vi "TestDriveEncoders.vi"(2 "WheelDiameter(in)":dbl=4.0, 3 "CountsPerRevolution":i32=4096, 4 "ZeroSensors":bool, 5 "RobotDriveMotors":T4[](array[typedef])) -> (0 "Drive Encoder Outputs":T3, 1 "Drive Encoder Outputs Raw":T1)   [LabVIEW 2017]
uses:
  <vilib>/Rock Robotics/WPI/MotorControl/WPI_MotorControlDeviceRef.ctl
  <vilib>/Rock Robotics/WPI/MotorControl/WPI_MotorControlType.ctl
  <vilib>/Rock Robotics/SystemInterfaces/DIO/FPGA_DIOPWMChannel.ctl
  <vilib>/Rock Robotics/WPI/PWM/WPI_PWMDeadband.ctl
  <vilib>/Rock Robotics/SystemInterfaces/DIO/FPGA_DIOChannel.ctl
  ArgosLib/Drive/MotorControl/TypeDefs/RobotDriveMotorSelectorEnum.ctl
  <vilib>/Rock Robotics/WPI/ThirdParty/Phoenix-LabVIEW/Motor Controller/Get/CTRE_Phoenix_MotorController_GetSelectedSensorData.vi
  ArgosLib/ArgosLib.lvlib
panel:
  out "Other Encoder Outputs":T2
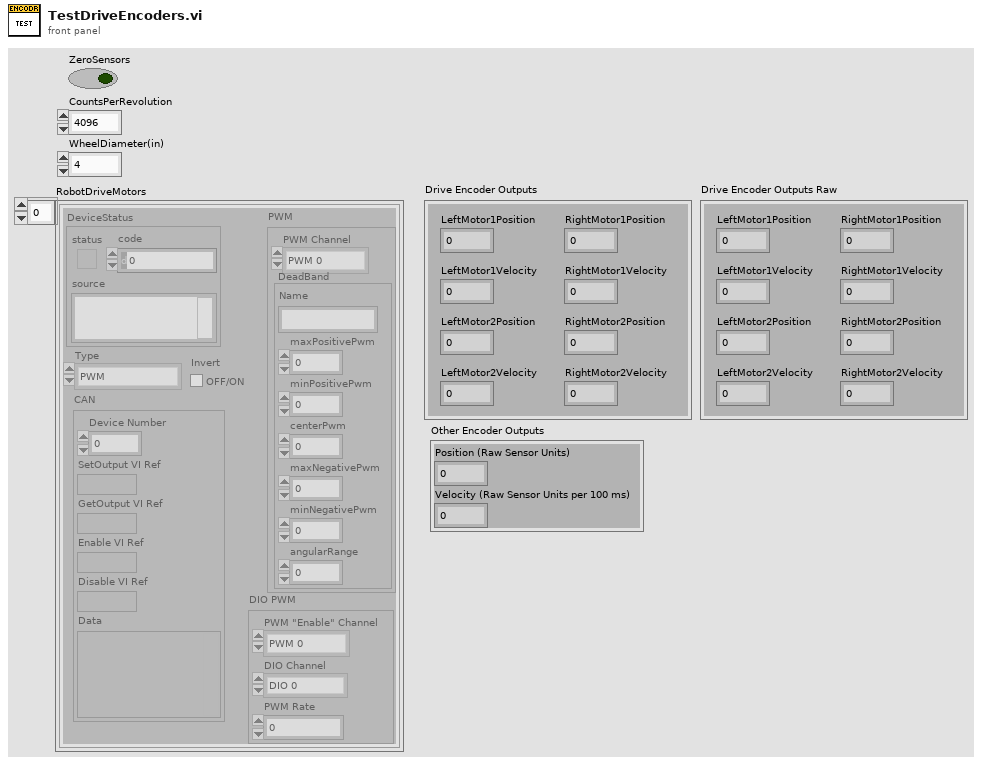
[diagram p1: front panel]
types:
  T1 = cluster{"LeftMotor1Position ":i32, "LeftMotor1Velocity":i32, "RightMotor1Velocity ":i32, "RightMotor1Position ":i32, "LeftMotor2Position ":i32, "LeftMotor2Velocity ":i32, "RightMotor2Position":i32, "RightMotor2Velocity":i32}
  T2 = cluster{"Position (Raw Sensor Units)":i32, "Velocity (Raw Sensor Units per 100 ms)":i32}
  T3 = cluster{"LeftMotor1Position ":dbl, "LeftMotor1Velocity":dbl, "RightMotor1Velocity ":dbl, "RightMotor1Position ":dbl, "LeftMotor2Position ":dbl, "LeftMotor2Velocity ":dbl, "RightMotor2Position":dbl, "RightMotor2Velocity":dbl}
  T4 = typedef "WPI_MotorControlDeviceRef.ctl" = cluster{"DeviceStatus":errorcluster, "Type":T5, "PWM":cluster{"PWM Channel":T6, "DeadBand":T7}, "CAN":cluster{"Device Number":u8, "SetOutput VI Ref":variant, "GetOutput VI Ref":variant, "Enable VI Ref":variant, "Disable VI Ref":variant, "Data":variant}, "Invert":bool, "DIO PWM":cluster{"PWM \"Enable\" Channel":T6, "DIOChannel":T8, "PWM Rate":dbl}}
  T5 = typedef "WPI_MotorControlType.ctl" = enum16{"PWM", "CAN", "DIO PWM"}
  T6 = typedef "FPGA_DIOPWMChannel.ctl" = enum8{"PWM 0", "PWM 1", "PWM 2", "PWM 3", "PWM 4", "PWM 5", "PWM 6", "PWM 7", "PWM 8", "PWM 9", "PWM MXP 0", "PWM MXP 1", "PWM MXP 2", "PWM MXP 3", "PWM MXP 4", "PWM MXP 5", "PWM MXP 6", "PWM MXP 7", "PWM MXP 8", "PWM MXP 9", "Invalid"}
  T7 = typedef "WPI_PWMDeadband.ctl" = cluster{"Name":string, "maxPositivePwm":i32, "minPositivePwm":i32, "centerPwm":i32, "maxNegativePwm":i32, "minNegativePwm":i32, "angularRange":u16}
  T8 = typedef "FPGA_DIOChannel.ctl" = enum8{"DIO 0", "DIO 1", "DIO 2", "DIO 3", "DIO 4", "DIO 5", "DIO 6", "DIO 7", "DIO 8", "DIO 9", "DIO MXP 0", "DIO MXP 1", "DIO MXP 2", "DIO MXP 3", "DIO MXP 4", "DIO MXP 5", "DIO MXP 6", "DIO MXP 7", "DIO MXP 8", "DIO MXP 9", "DIO MXP 10", "DIO MXP 11", "DIO MXP 12", "DIO MXP 13", "DIO MXP 14", "DIO MXP 15", "SPI Port CS1", "SPI Port CS2", "SPI Port CS3", "SPI Port MISO", "SPI Port MOSI", "Invalid"}
  T9 = typedef "ArgosLib.lvlib/RobotDriveMotorSelectorEnum.ctl" = enum16{"Left Motor 1", "Right Motor 1", "Left Motor 2", "Right Motor 2", "Left Motor 3", "Right Motor 3"}
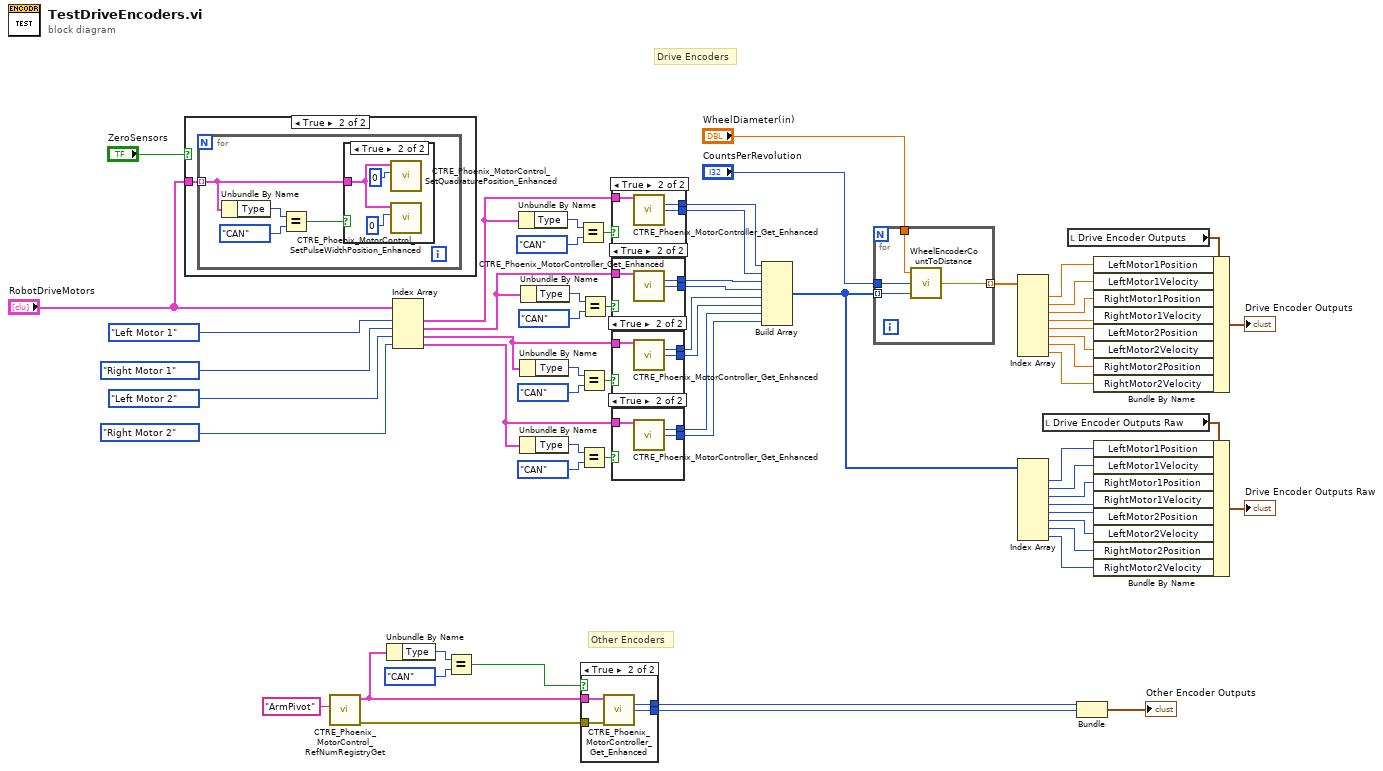
[diagram p0: block diagram]
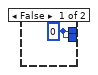
[diagram p2: hidden frame]
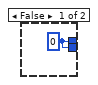
[diagram p3: hidden frame]
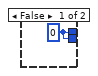
[diagram p4: hidden frame]
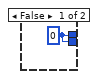
[diagram p5: hidden frame]
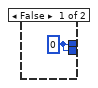
[diagram p6: hidden frame]
diagram:
  # "Other Encoders"
  # "Drive Encoders"
  n1 = case shown="True" "ZeroSensors" {
    tunnel: "RobotDriveMotors" -> [_ w64]
    frame False {
    }
    frame True {
      n2 = for {
        tunnel: w64 -> [w68] mode=indexing
        n3 = Unbundle By Name(w68) -> ("Type"=w67:T5)
        n4 = Equal?(x=w67, y=WPI_MotorControlType."CAN" ("Type")) -> (x = y?=w65:bool)
        n5 = case shown="True" w65 {
          tunnel: w68 -> [_ w69]
          frame False {
          }
          frame True {
            n6 = call <vilib>:"CTRE_Phoenix_MotorControl_SetQuadraturePosition_Enhanced.vi"("New Position"=0, "PhoenixMotorControlDevRef"=w69) -> ()  [unwired: 8 in, 2 out]
            n7 = call <vilib>:"CTRE_Phoenix_MotorControl_SetPulseWidthPosition_Enhanced.vi"("New Position"=0, "PhoenixMotorControlDevRef"=w69) -> ()  [unwired: 8 in, 2 out]
          }
        }
      }
    }
  }
  n8 = call <vilib>:"CTRE_Phoenix_MotorControl_RefNumRegistryGet.vi"("refnum name"="ArmPivot") -> ("error out"=w37:errorcluster, "PhoenixMotorControlDevRef"=w18:T4)  [unwired: 9 in]
  n9 = Unbundle By Name(w18) -> ("Type"=w19:T5)
  n10 = Index Array(array="RobotDriveMotors", index #1=RobotDriveMotorSelectorEnum."Left Motor 1" ("Motor Selector Enum"), index #2=RobotDriveMotorSelectorEnum."Right Motor 1" ("Motor Selector Enum"), index #3=RobotDriveMotorSelectorEnum."Left Motor 2" ("Motor Selector Enum"), index #4=RobotDriveMotorSelectorEnum."Right Motor 2" ("Motor Selector Enum")) -> (element #1=w8:T4, element #2=w7:T4, element #3=w6:T4, element #4=w5:T4)
  n11 = Equal?(x=w19, y=WPI_MotorControlType."CAN" ("Type")) -> (x = y?=w17:bool)
  n12 = Unbundle By Name(w8) -> ("Type"=w16:T5)
  n13 = Unbundle By Name(w6) -> ("Type"=w12:T5)
  n14 = Unbundle By Name(w5) -> ("Type"=w9:T5)
  n15 = Unbundle By Name(w7) -> ("Type"=w13:T5)
  n16 = Equal?(x=w16, y=WPI_MotorControlType."CAN" ("Type")) -> (x = y?=w1:bool)
  n17 = Equal?(x=w12, y=WPI_MotorControlType."CAN" ("Type")) -> (x = y?=w3:bool)
  n18 = Equal?(x=w9, y=WPI_MotorControlType."CAN" ("Type")) -> (x = y?=w4:bool)
  n19 = Equal?(x=w13, y=WPI_MotorControlType."CAN" ("Type")) -> (x = y?=w2:bool)
  n20 = case shown="True" w17 {
    tunnel: w37 -> [_ w76]
    tunnel: [w72 w75] -> w36
    tunnel: [w72 w74] -> w35
    tunnel: w18 -> [_ w73]
    frame False {
      w72 = 0 ("Position (Raw Sensor Units)")
    }
    frame True {
      n21 = call-poly <vilib>:"CTRE_Phoenix_MotorController_Get_Enhanced.vi"("PhoenixMotorControlDevRef"=w73, "error in"=w76) -> ("Position (Raw Sensor Units)"=w75:i32, "Velocity (Raw Sensor Units per 100 ms)"=w74:i32)  [unwired: 10 in, 2 out]
    }
  }
  n22 = case shown="True" w1 {
    tunnel: w8 -> [_ w80]
    tunnel: [w77 w79] -> w59
    tunnel: [w77 w78] -> w58
    frame False {
      w77 = 0 ("Position (Raw Sensor Units)")
    }
    frame True {
      n23 = call-poly <vilib>:"CTRE_Phoenix_MotorController_Get_Enhanced.vi"("PhoenixMotorControlDevRef"=w80) -> ("Position (Raw Sensor Units)"=w79:i32, "Velocity (Raw Sensor Units per 100 ms)"=w78:i32)  [unwired: 11 in, 2 out]
    }
  }
  n24 = case shown="True" w2 {
    tunnel: w7 -> [_ w84]
    tunnel: [w81 w83] -> w53
    tunnel: [w81 w82] -> w52
    frame False {
      w81 = 0 ("Position (Raw Sensor Units)")
    }
    frame True {
      n25 = call-poly <vilib>:"CTRE_Phoenix_MotorController_Get_Enhanced.vi"("PhoenixMotorControlDevRef"=w84) -> ("Position (Raw Sensor Units)"=w83:i32, "Velocity (Raw Sensor Units per 100 ms)"=w82:i32)  [unwired: 11 in, 2 out]
    }
  }
  n26 = case shown="True" w3 {
    tunnel: w6 -> [_ w88]
    tunnel: [w85 w87] -> w57
    tunnel: [w85 w86] -> w56
    frame False {
      w85 = 0 ("Position (Raw Sensor Units)")
    }
    frame True {
      n27 = call-poly <vilib>:"CTRE_Phoenix_MotorController_Get_Enhanced.vi"("PhoenixMotorControlDevRef"=w88) -> ("Position (Raw Sensor Units)"=w87:i32, "Velocity (Raw Sensor Units per 100 ms)"=w86:i32)  [unwired: 11 in, 2 out]
    }
  }
  n28 = case shown="True" w4 {
    tunnel: w5 -> [_ w92]
    tunnel: [w89 w91] -> w55
    tunnel: [w89 w90] -> w54
    frame False {
      w89 = 0 ("Position (Raw Sensor Units)")
    }
    frame True {
      n29 = call-poly <vilib>:"CTRE_Phoenix_MotorController_Get_Enhanced.vi"("PhoenixMotorControlDevRef"=w92) -> ("Position (Raw Sensor Units)"=w91:i32, "Velocity (Raw Sensor Units per 100 ms)"=w90:i32)  [unwired: 11 in, 2 out]
    }
  }
  n30 = Build Array(w59, w58, w53, w52, w57, w56, w55, w54) -> (w22:i32[])
  n31 = for {
    tunnel: w22 -> [w96] mode=indexing
    tunnel: [w95] -> w51 mode=indexing
    tunnel: "CountsPerRevolution" -> [w94]
    tunnel: "WheelDiameter(in)" -> [w93]
    n32 = call "WheelEncoderCountToDistance.vi"("EncoderCounts"=w96, "CountsPerRevolution"=w94, "WheelDiameter(in)"=w93) -> ("Output(in)"=w95:dbl)
  }
  n33 = Index Array(array=w51) -> (element #1=w45:dbl, element #2=w44:dbl, element #3=w43:dbl, element #4=w42:dbl, element #5=w41:dbl, element #6=w40:dbl, element #7=w39:dbl, element #8=w38:dbl)  [unwired: 8 in]
  n34 = Index Array(array=w22) -> (element #1=w23:i32, element #2=w24:i32, element #3=w25:i32, element #4=w26:i32, element #5=w27:i32, element #6=w28:i32, element #7=w29:i32, element #8=w30:i32)  [unwired: 8 in]
  n35 = local read "Drive Encoder Outputs Raw"() -> (w31:T1)
  n36 = local read "Drive Encoder Outputs"() -> (w32:T3)
  n37 = Bundle("Position (Raw Sensor Units)"=w36, "Velocity (Raw Sensor Units per 100 ms)"=w35) -> (→"Other Encoder Outputs":T2)  [unwired: 1 in]
  n38 = Bundle By Name(cluster=w32, "LeftMotor1Position"=w45, "LeftMotor1Velocity"=w44, "RightMotor1Position"=w43, "RightMotor1Velocity"=w42, "LeftMotor2Position"=w41, "LeftMotor2Velocity"=w40, "RightMotor2Position"=w39, "RightMotor2Velocity"=w38) -> (→"Drive Encoder Outputs":T3)
  n39 = Bundle By Name(cluster=w31, "LeftMotor1Position"=w23, "LeftMotor1Velocity"=w24, "RightMotor1Position"=w25, "RightMotor1Velocity"=w26, "LeftMotor2Position"=w27, "LeftMotor2Velocity"=w28, "RightMotor2Position"=w29, "RightMotor2Velocity"=w30) -> (→"Drive Encoder Outputs Raw":T1)
